vi "RT_Servo_Controller_Loop.vi"(8 "error in (no error)":errorcluster={"status"=FALSE, "code"=0, "source"="\"\""}, 10 "encoder data":string, 11 "Setpoint/mode":string) -> (0 "error out":errorcluster={"status"=FALSE, "code"=0, "source"="\"\""}, 2 "status ok":bool, 3 "Servo feedback/health":string)   [LabVIEW 2026]
doc: "INTENT: Control PC lever position. LOGIC: In fixed-rate service accept authorized motion target, enforce motion limit/profile, read encoder and track errors."
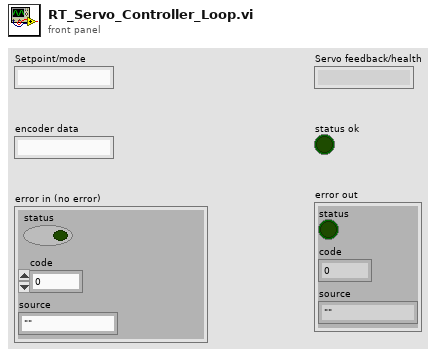
[diagram p1: front panel]
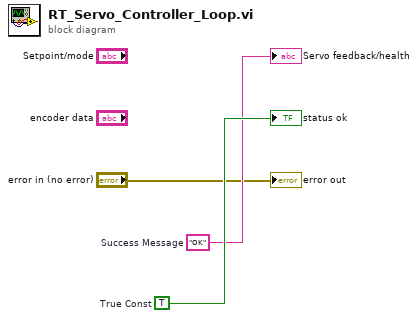
[diagram p0: block diagram]
diagram:
  w3 = TRUE  # True Const
  w2 = "OK"  # Success Message
  "Servo feedback/health" <- w2
  "status ok" <- w3
  "error out" <- "error in (no error)"
